vi "RemoteVI Splitter Request.vi"(0 "put?":bool, 1 "hWnd":u64, 2 "id":u64, 3 "pos":i32) -> (4 "pending?":bool, 5 "id out":u64, 6 "pos out":i32)   [LabVIEW 2020, in "RemoteVI.lvlib"]
doc: "Keeps the splitter move a client asked for (s id pos, docs\\protocol.md section 4) until the server loop may make VI Server calls - a functional global (a Feedback Node outside any loop, initialized on the first call only, so the state survives between calls of this non-reentrant VI). put? TRUE (RemoteVI Handle Text Message.vi) stores id and pos for the panel hWnd, replacing a move not applied yet. put? FALSE (RemoteVI Apply Splitter.vi) takes the move stored for hWnd: pending? is TRUE and id out, pos out are the move, which is then forgotten; a move stored for another panel (another server of this LabVIEW instance) stays. One slot: the moves of two servers within one loop iteration keep the later one. Pure G, no I/O."
uses:
  RemoteVI.lvlib
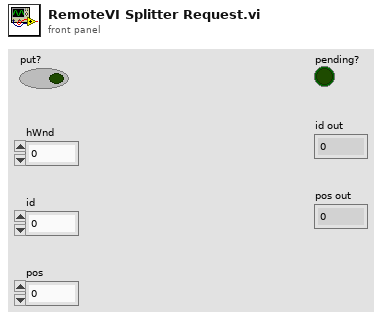
[diagram p1: front panel]
types:
  T1 = cluster{"valid":bool, "hWnd":u64, "id":u64, "pos":i32}
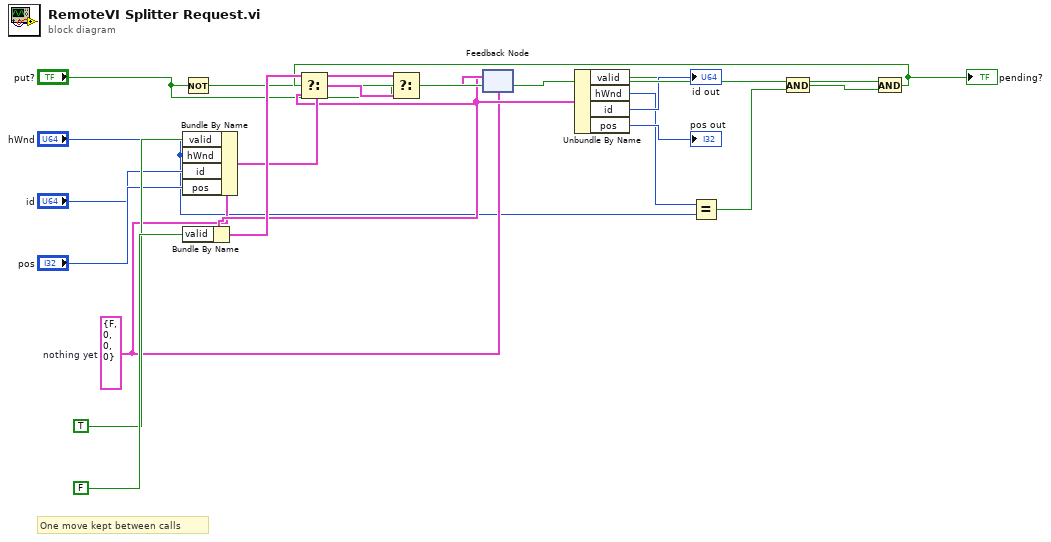
[diagram p0: block diagram]
diagram:
  w5 = T1 {"valid"=FALSE, "hWnd"=0, "id"=0, "pos"=0}  # nothing yet
  # "One move kept between calls"
  n1 = Not(x="put?") -> (.not. x?=w14:bool)
  n2 = Bundle By Name(cluster=w5, "valid"=TRUE, "hWnd"="hWnd", "id"="id", "pos"="pos") -> (w18:T1)
  n3 = feedback #1(w5) -> (w6:T1)
  n4 = Bundle By Name(cluster=w6, "valid"=FALSE) -> (w19:T1)
  n5 = Unbundle By Name(w6) -> ("valid"=w8:bool, "hWnd"=w9:u64, "id"=→"id out":u64, "pos"=→"pos out":i32)
  n6 = Equal?(x=w9, y="hWnd") -> (x = y?=w12:bool)
  n7 = And(x=w8, y=w12) -> (x .and. y?=w13:bool)
  n8 = And(x=w14, y=w13) -> (x .and. y?=w15:bool)
  "pending?" <- w15
  n9 = Select(t=w19, s=w15, f=w6) -> (s? t:f=w20:T1)
  n10 = Select(t=w18, s="put?", f=w20) -> (s? t:f=w7:T1)
  n11 = feedback-in #1(w7) -> ()
